vi "Build Source Waveform.vi"(0 "RFFE Command in":refnum<class "RFFE Command.lvclass">, 11 "error in (no error)":errorcluster) -> (4 "RFFE Command out":refnum<class "RFFE Command.lvclass">, 6 "Source Waveform":u32[](array[numeric]), 15 "error out":errorcluster)   [LabVIEW 2018, in "MIPI RFFE API.lvlib" / "RFFE Command.lvclass"]
uses:
  RFFE Command.lvclass
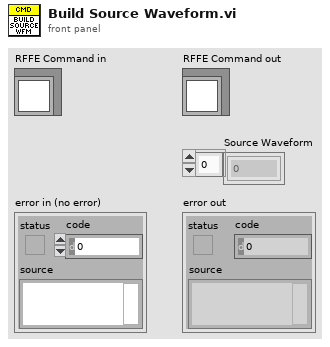
[diagram p1: front panel]
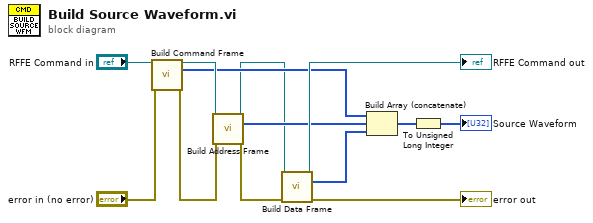
[diagram p0: block diagram]
diagram:
  n1 = call-dynamic "Build Command Frame.vi"("RFFE Command in"="RFFE Command in", "error in (no error)"="error in (no error)") -> ("RFFE Command out"=w8:refnum<class "RFFE Command.lvclass">, "Command Frame"=w7:u8[], "error out"=w1:errorcluster)  [unwired: 11 in]
  n2 = call-dynamic "Build Address Frame.vi"("RFFE Command in"=w8, "error in (no error)"=w1) -> ("RFFE Command out"=w4:refnum<class "RFFE Command.lvclass">, "Address Frame"=w6:u8[], "error out"=w3:errorcluster)  [unwired: 11 in]
  n3 = call-dynamic "Build Data Frame.vi"("RFFE Command in"=w4, "error in (no error)"=w3) -> ("RFFE Command out"=→"RFFE Command out":refnum<class "RFFE Command.lvclass">, "Data Frame"=w2:u8[], "error out"=→"error out":errorcluster)  [unwired: 11 in]
  n4 = Build Array (concatenate)(w7, w6, w2) -> (w5:u8[])
  n5 = To Unsigned Long Integer(number=w5) -> (unsigned 32bit integer=→"Source Waveform":u32[])
